vi "Launch.vi"(8 "error in (no error)":errorcluster, 10 "NavigatorEvents":T1, 11 "NavigatableView in":refnum<class "NavigatableView.lvclass">) -> (0 "error out":errorcluster, 2 "VIReference":refnum<vi>, 3 "NavigatableView out":refnum<class "NavigatableView.lvclass">)   [LabVIEW 2024, in "NavigatableView.lvclass"]
doc: "Create stop event and launch view asynchronously.\n\nNavigatorEvents - used to navigate the app from inside a view's viewmodel. Do this by generating the relevant event (go, push, pop) and if necessary, pass in the route name (setup when Navigator is initialised).\n\nVIReference - this should output the VI reference of the view (UI) that has been launched. To launch a view, wire up the following: strictly typed Static VI Reference > Property Node (VI Path) > Open VI Reference > Start Asynchronous Call"
uses:
  NavigatableView.lvclass
  Navigator/NavigatorEvents.ctl
  NavigatableView.lvclass/NavigatableView.ctl
  Navigator/Navigator.lvclass
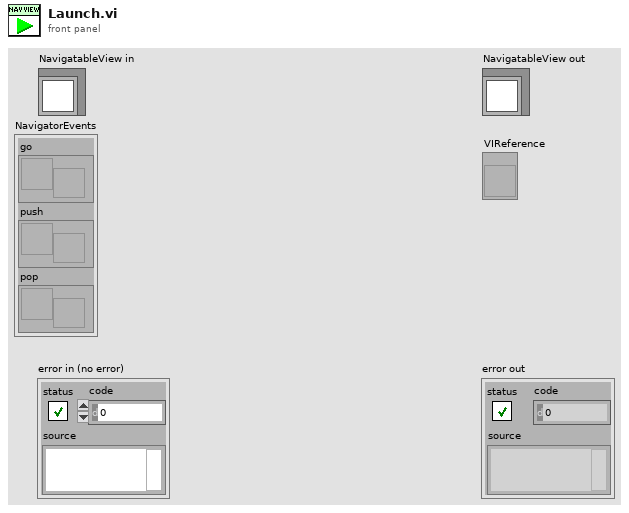
[diagram p1: front panel]
types:
  T1 = typedef "Navigator.lvclass/NavigatorEvents.ctl" = cluster{"go":refnum<user-event>, "push":refnum<user-event>, "pop":refnum<user-event>}
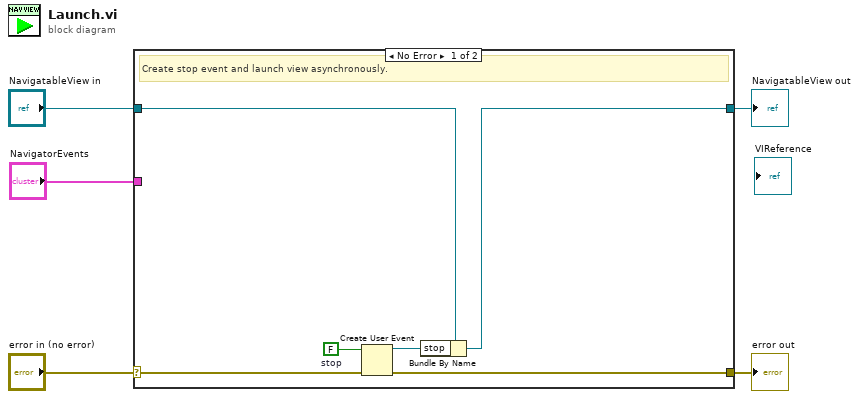
[diagram p0: block diagram]
diagram:
  n1 = case shown="No Error" "error in (no error)" {
    selector: "error in (no error)" -> [w10 w13]
    tunnel: [w9 w13] -> w4
    tunnel: [w7 w12] -> w2
    tunnel: "NavigatableView in" -> [w8 w12]
    tunnel: "NavigatorEvents" -> [_ _]
    frame No Error {
      w11 = FALSE  # stop
      # "Create stop event and launch view asynchronously."
      n2 = Create User Event(user event datatype=w11, error in=w10) -> (user event=w6:refnum<user-event>, error out=w9:errorcluster)
      n3 = Bundle By Name(cluster=w8, "stop"=w6) -> (w7:refnum<class "NavigatableView.lvclass">)
    }
    frame Error {
    }
  }
  "error out" <- w4
  "NavigatableView out" <- w2
